vi "FPGA Main.vi"   [LabVIEW 2013]
uses:
  dynamic profibus/profibus master action.ctl
  dynamic profibus/profibus master transmit header.ctl
  dynamic profibus/error enum.ctl
  <vilib>/rvi/eio/common/nirviEmuTemplatePropertySet_errors.vi
  <vilib>/rvi/Emulation/niFpgaSctlEmulationGetInTimedLoop.vi
  <vilib>/rvi/Emulation/niFpgaEmulationReportErrorSimple.vi
  <vilib>/rvi/Emulation/niFpgaGetClockAttributes.vi
  <vilib>/rvi/DataTransferAndStorage/Container/Common/niFpgaContainerExecOnDevCompGetState.vi
  <vilib>/rvi/FIFO/Fifo_Resource/nirvififoEmulationReadFpgaImpl.vi
  <vilib>/rvi/DataTransferAndStorage/Container/Common/niFpgaContainerGetUniqueNameForEmu.vi
  <vilib>/rvi/interface/RandomDataEmulation/nirviRandomDataFPGAFIFO.vi
  <vilib>/rvi/interface/RandomDataEmulation/niFpgaRandomDataHandleErrors.vi
  <vilib>/rvi/eio/common/nirviEmuReportErrorAndStop.vi
  <vilib>/rvi/eio/common/nirviEmuTemplateMethod_errors.vi
  <vilib>/rvi/FIFO/Fifo_Resource/nirvififoEmulationWriteFpgaImpl.vi
  <vilib>/rvi/Emulation/niFpgaCriticalErrorInLSC.vi
  <vilib>/eio/EIOPropertyNode/EIOPropertyNode.xnode
  <vilib>/rvi/DataTransferAndStorage/Container/XNode/niFpgaContainer.xnode
  <vilib>/rvi/FIFO/Fifo_Resource/niFpgaFifoEmulationRefIn.vi
  <vilib>/eio/EIOMethodNode/EIOMethodNode.xnode
  <vilib>/rvi/eio/common/nirviEmuTemplatePropertyGet_errors.vi
  <vilib>/rvi/eio/common/nirviEmuTemplatePropertyGet_noerrors.vi
  <vilib>/rvi/eio/common/nirviEmuTemplatePropertySet_noerrors.vi
  dynamic profibus/dynamic profibus.lvlib
  <vilib>/rvi/LocalResourceManager/LocalResourceManager.xnode
  <vilib>/rvi/DataTransferAndStorage/Register/Emulation/niFpgaRegisterEmulationRefIn.vi
  <vilib>/rvi/DataTransferAndStorage/Container/Common/niFpgaContainerSetEmuInfo.vi
  <vilib>/rvi/DataTransferAndStorage/Register/Emulation/niFpgaRegisterEmulation.vi
types:
  T1 = typedef "dynamic profibus.lvlib/profibus master action.ctl" = enum8{"initialize", "uninitialize", "stop", "get input", "get input size", "set output", "get output size", "get diagnostic", "transfer data", "transfer diagnostics", "read many inputs"}
  T2 = typedef "dynamic profibus.lvlib/profibus master transmit header.ctl" = enum8{"Error", "Input", "Diagnostic", "input size", "output size", "many inputs"}
  T3 = typedef "dynamic profibus.lvlib/error enum.ctl" = u16
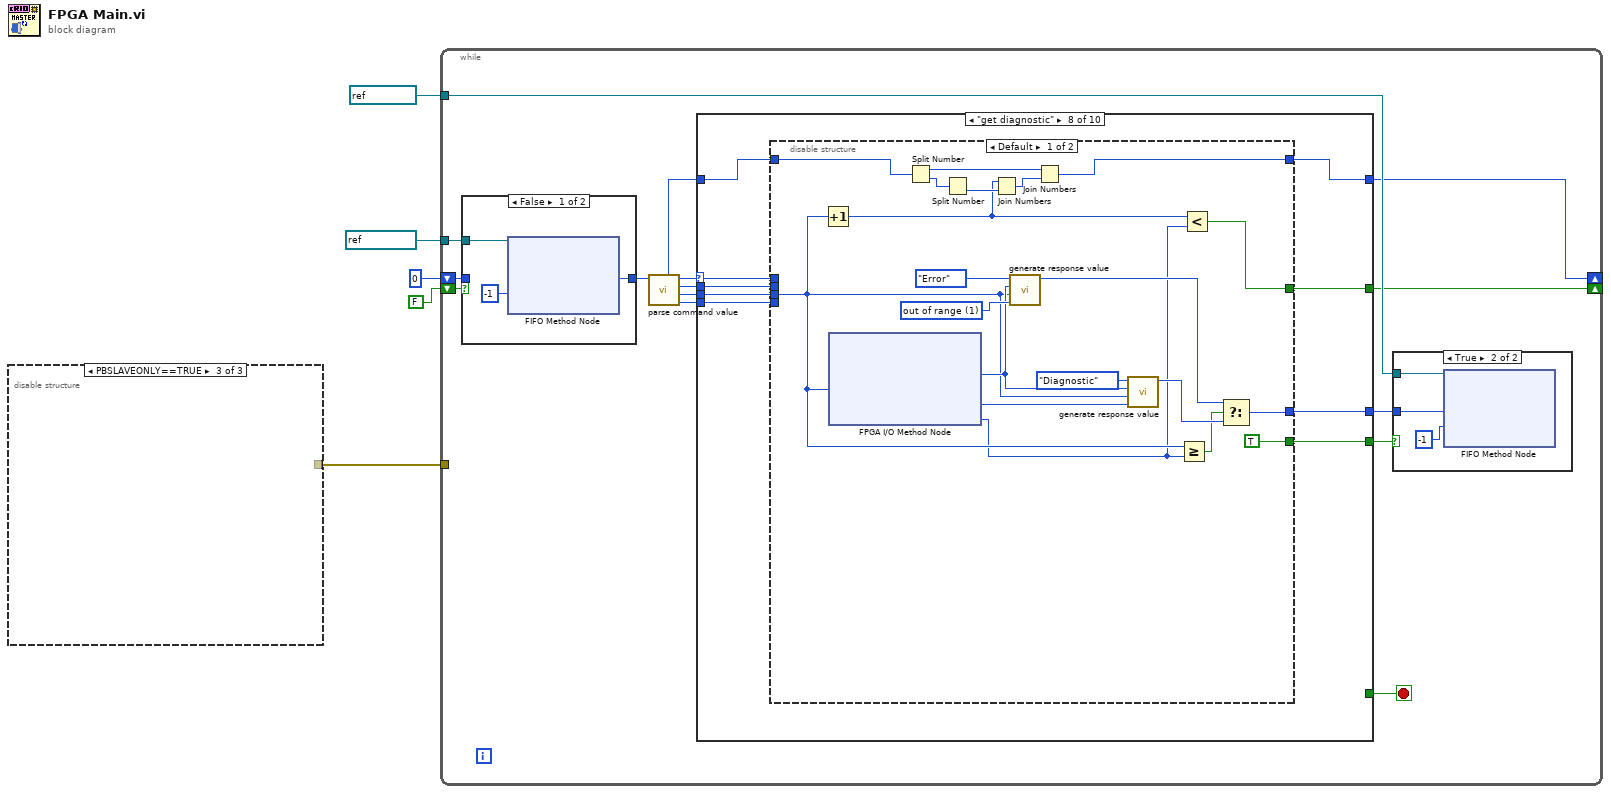
[diagram p0: block diagram]
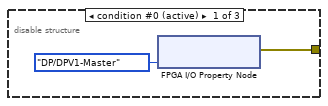
[diagram p2: hidden frame]
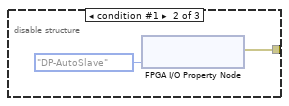
[diagram p3: hidden frame]
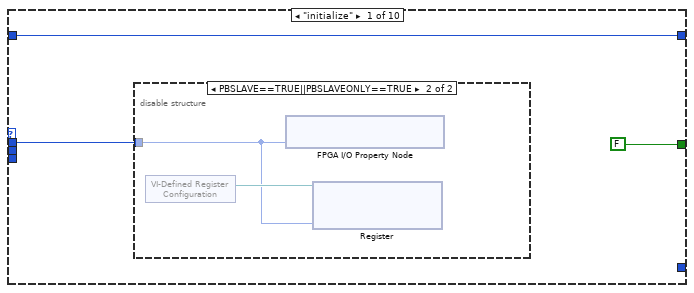
[diagram p6: hidden frame]
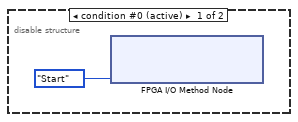
[diagram p7: hidden frame]
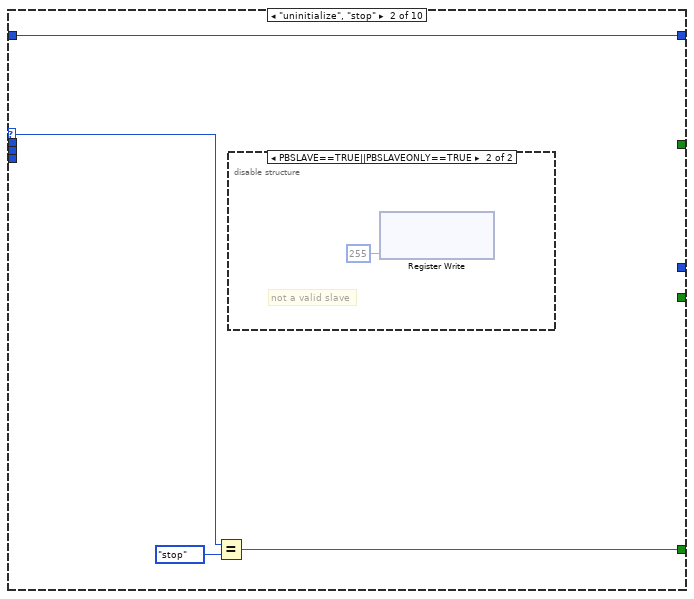
[diagram p8: hidden frame]
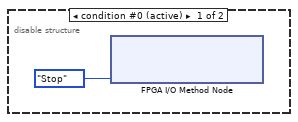
[diagram p9: hidden frame]
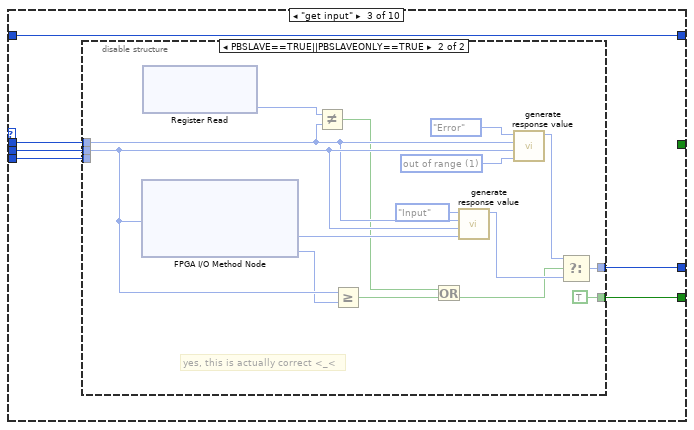
[diagram p10: hidden frame]
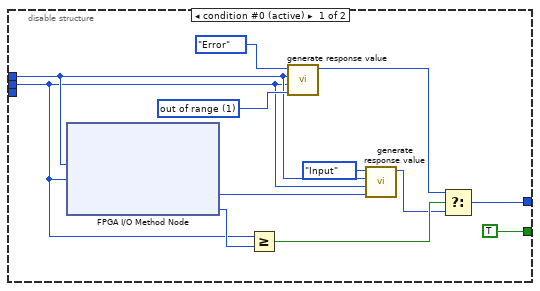
[diagram p11: hidden frame]
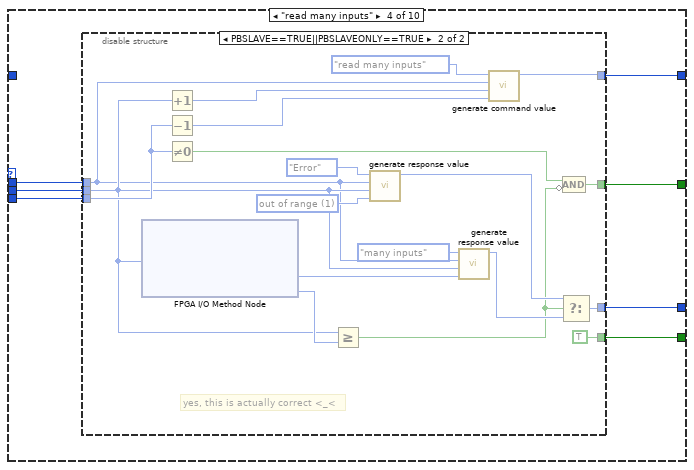
[diagram p12: hidden frame]
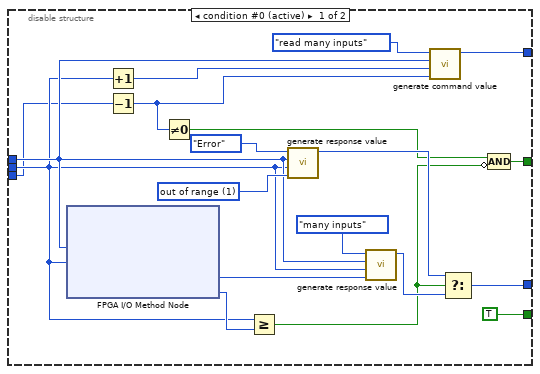
[diagram p13: hidden frame]
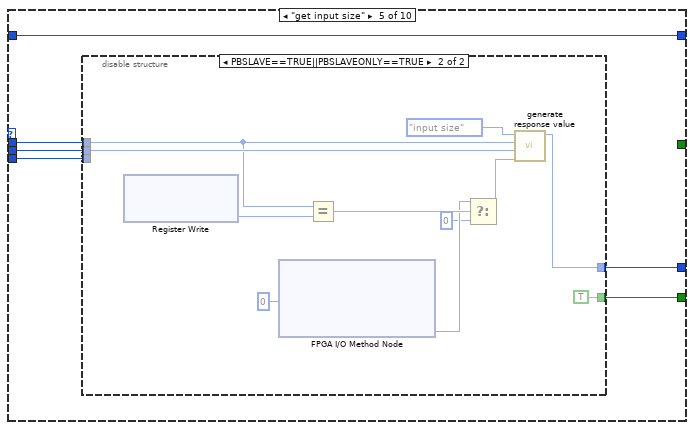
[diagram p14: hidden frame]
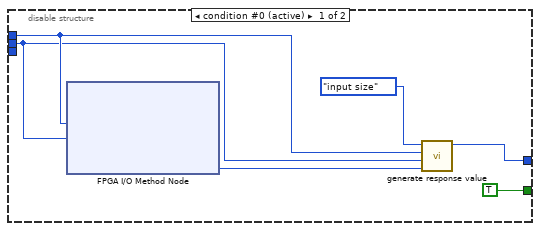
[diagram p15: hidden frame]
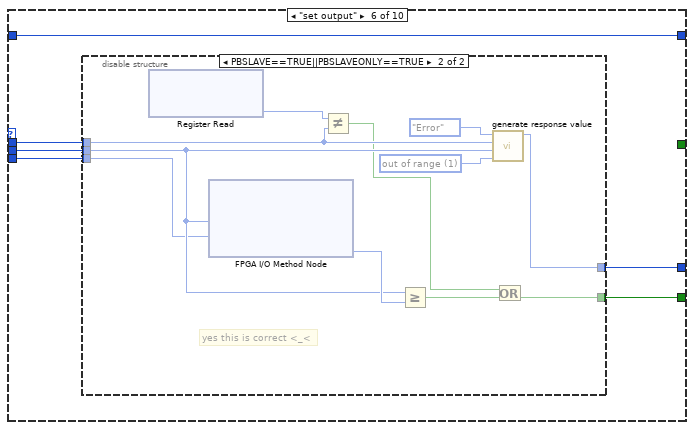
[diagram p16: hidden frame]
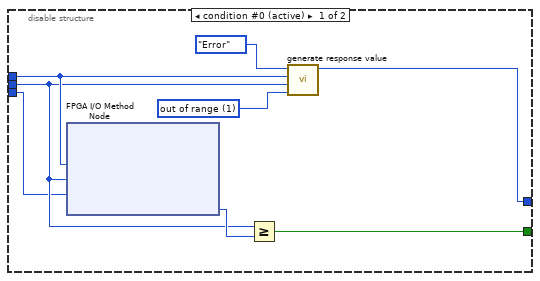
[diagram p17: hidden frame]
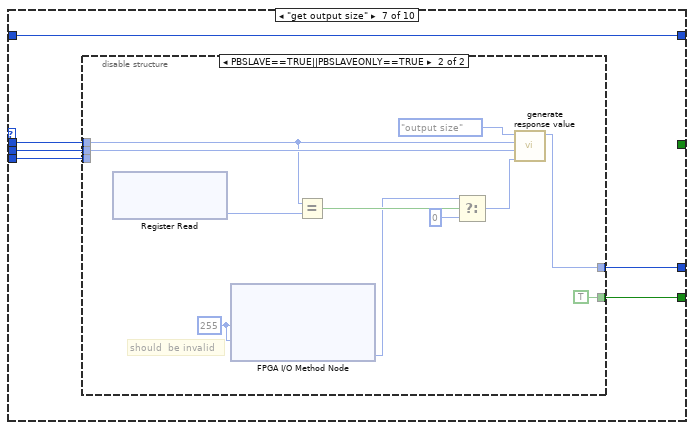
[diagram p18: hidden frame]
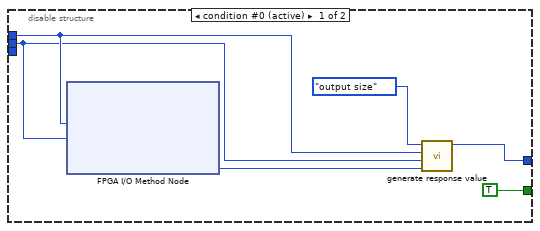
[diagram p19: hidden frame]
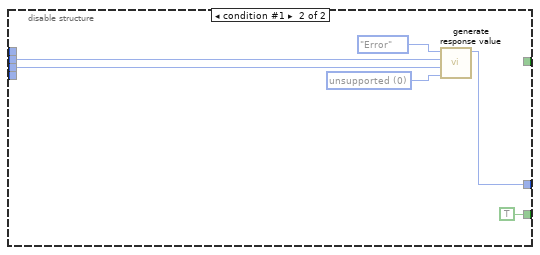
[diagram p20: hidden frame]
diagram:
  n1 = disable-structure shown="PBSLAVEONLY==TRUE" {
    disable-tunnel: [w6 w8 _] -> w3
    frame condition #0 (active) {
      n2 = xnode "FPGA I/O Property Node"("Init cRIO PB"=enum8{"DP/DPV1-Master", "DP-AutoSlave"}."DP/DPV1-Master" ("Start-up cRIO PB")) -> ("error out"=w6:errorcluster)  [unwired: 2 in, 1 out]
    }
    frame condition #1 {
      n3 = xnode "FPGA I/O Property Node"("Init cRIO PB"=enum8{"DP/DPV1-Master", "DP-AutoSlave"}."DP-AutoSlave" ("Start-up cRIO PB")) -> ("error out"=w8:errorcluster)  [unwired: 2 in, 1 out]
    }
    frame condition #2 {
    }
  }
  n4 = while {
    tunnel: refnum<k21> "ToFPGA" ("FIFO In") -> [w23]
    tunnel: refnum<k21> "ToHost" ("FIFO In") -> [w22]
    tunnel: w3 -> [_]
    shift-right: [w10] -> _
    shift-left: FALSE -> [w13]
    shift-right: [w11] -> _
    shift-left: u32 0 ("full element") -> [w12]
    stop <- w24 stop-if-true
    n5 = case shown="False" w13 {
      tunnel: w23 -> [w27 _]
      tunnel: [w26 w28] -> w21
      tunnel: w12 -> [_ w28]
      frame False {
        n6 = xnode ("FIFO Method Node")("Timeout"=-1, "FIFO In"=w27) -> ("Element"=w26:u32)  [unwired: 2 out]
      }
      frame True {
      }
    }
    n7 = call "parse command value.vi"("Element"=w21) -> ("data"=w17:u8, "index"=w18:u8, "device"=w19:u8, "action"=w20:T1, "full element"=w16:u32)  [unwired: 6 in]
    n8 = case shown="\"get diagnostic\"" w20 {
      selector: w20 -> [_ w41 _ _ _ _ _ w195 _ _]
      tunnel: w19 -> [w34 _ w45 w79 w123 w146 w171 w197 w229 w250]
      tunnel: w18 -> [_ _ w49 w83 w127 w150 w175 w201 w233 w254]
      tunnel: w17 -> [_ _ w48 w82 w126 w149 w174 w200 w232 w253]
      tunnel: w16 -> [w33 w38 w44 _ w122 w145 w170 w196 w228 w249]
      tunnel: [_ _ w47 w81 w125 w148 w173 w199 w231 w252] -> w15
      tunnel: [_ _ w46 w80 w124 w147 w172 w198 w230 w251] -> w14
      tunnel: [_ w39 _ _ _ _ _ _ _ _] -> w24
      tunnel: [w33 w38 w44 w78 w122 w145 w170 w194 w228 w249] -> w11
      tunnel: [FALSE _ _ w77 _ _ _ w193 _ _] -> w10
      frame "initialize" {
        n9 = disable-structure shown="PBSLAVE==TRUE||PBSLAVEONLY==TRUE" {
          disable-tunnel: w34 -> [_ w36]
          frame condition #0 (active) {
            n10 = xnode "FPGA I/O Method Node"("Mode"=enum16{"Start", "Stop"}."Start") -> ()  [unwired: 2 in, 2 out]
          }
          frame condition #1 {
            n11 = xnode ("VI-Defined Register Configuration")() -> ("Register Out"=w37:refnum<k21>)
            n12 = xnode "FPGA I/O Property Node"("DP-AutoSlave Address"=w36) -> ()  [unwired: 2 in, 2 out]
            n13 = xnode "Register"("Data"=w36, "Register In"=w37) -> ()  [unwired: 1 out]
          }
        }
      }
      frame "uninitialize", "stop" {
        n14 = Equal?(x=w41, y=profibus_master_action."stop") -> (x = y?=w39:bool)
        n15 = disable-structure shown="PBSLAVE==TRUE||PBSLAVEONLY==TRUE" {
          frame condition #0 (active) {
            n16 = xnode "FPGA I/O Method Node"("Mode"=enum16{"Start", "Stop"}."Stop") -> ()  [unwired: 2 in, 2 out]
          }
          frame condition #1 {
            # "not a valid slave"
            n17 = xnode "Register Write"("Data"=u8 255) -> ()  [unwired: 1 in, 1 out]
          }
        }
      }
      frame "get input" {
        n18 = disable-structure shown="PBSLAVE==TRUE||PBSLAVEONLY==TRUE" {
          disable-tunnel: w49 -> [w51 w67]
          disable-tunnel: w48 -> [_ _]
          disable-tunnel: [TRUE TRUE] -> w47
          disable-tunnel: [w55 w68] -> w46
          disable-tunnel: w45 -> [w52 w64]
          frame condition #0 (active) {
            w59 = T3 1 items=["unsupported", "out of range"]
            n19 = xnode "FPGA I/O Method Node"("Slave"=w52, "Index"=w51) -> ("Data"=w53:u8, "Length"=w58:u8)  [unwired: 1 in, 1 out]
            n20 = Greater Or Equal?(x=w51, y=w58) -> (x >= y?=w57:bool)
            n21 = call "generate response value.vi"("data"=w59, "index"=w51, "device"=w52, "header"=profibus_master_transmit_header."Error") -> ("Element"=w56:u32)  [unwired: 7 in]
            n22 = call "generate response value.vi"("data"=w53, "index"=w51, "device"=w52, "header"=profibus_master_transmit_header."Input") -> ("Element"=w54:u32)  [unwired: 7 in]
            n23 = Select(t=w56, s=w57, f=w54) -> (s? t:f=w55:u32)
          }
          frame condition #1 {
            w71 = T3 1 items=["unsupported", "out of range"]
            # "yes, this is actually correct <_<"
            n24 = xnode "FPGA I/O Method Node"("Index"=w67) -> ("Data"=w72:u8, "Length"=w66:u8)  [unwired: 1 in, 1 out]
            n25 = xnode "Register Read"() -> ("Data"=w63:u8)  [unwired: 1 in, 1 out]
            n26 = Not Equal?(x=w63, y=w64) -> (x != y?=w62:bool)
            n27 = Greater Or Equal?(x=w67, y=w66) -> (x >= y?=w75:bool)
            n28 = Or(x=w62, y=w75) -> (x .or. y?=w65:bool)
            n29 = call "generate response value.vi"("data"=w72, "index"=w67, "device"=w64, "header"=profibus_master_transmit_header."Input") -> ("Element"=w76:u32)  [unwired: 7 in]
            n30 = call "generate response value.vi"("data"=w71, "index"=w67, "device"=w64, "header"=profibus_master_transmit_header."Error") -> ("Element"=w74:u32)  [unwired: 7 in]
            n31 = Select(t=w74, s=w65, f=w76) -> (s? t:f=w68:u32)
          }
        }
      }
      frame "read many inputs" {
        n32 = disable-structure shown="PBSLAVE==TRUE||PBSLAVEONLY==TRUE" {
          disable-tunnel: w83 -> [w90 w106]
          disable-tunnel: w82 -> [w87 w107]
          disable-tunnel: [TRUE TRUE] -> w81
          disable-tunnel: [w97 w114] -> w80
          disable-tunnel: w79 -> [w91 w105]
          disable-tunnel: [w93 w108] -> w78
          disable-tunnel: [w85 w104] -> w77
          frame condition #0 (active) {
            w100 = T3 1 items=["unsupported", "out of range"]
            n33 = xnode "FPGA I/O Method Node"("Slave"=w91, "Index"=w90) -> ("Data"=w95:u8, "Length"=w99:u8)  [unwired: 1 in, 1 out]
            n34 = Increment(x=w90) -> (x+1=w89:u8)
            n35 = Decrement(x=w87) -> (x-1=w84:u8)
            n36 = Not Equal To 0?(x=w84) -> (x != 0?=w86:bool)
            n37 = Greater Or Equal?(x=w90, y=w99) -> (x >= y?=w88:bool)
            n38 = call "generate response value.vi"("data"=w100, "index"=w90, "device"=w91, "header"=profibus_master_transmit_header."Error") -> ("Element"=w98:u32)  [unwired: 7 in]
            n39 = call "generate response value.vi"("data"=w95, "index"=w90, "device"=w91, "header"=profibus_master_transmit_header."many inputs") -> ("Element"=w96:u32)  [unwired: 7 in]
            n40 = call "generate command value.vi"("data"=w84, "index"=w89, "device"=w91, "action"=profibus_master_action."read many inputs") -> ("Element"=w93:u32)  [unwired: 7 in]
            n41 = Select(t=w98, s=w88, f=w96) -> (s? t:f=w97:u32)
            n42 = Compound Arithmetic op=AND(w86, invert w88) -> (w85:bool)
          }
          frame condition #1 {
            w117 = T3 1 items=["unsupported", "out of range"]
            # "yes, this is actually correct <_<"
            n43 = xnode "FPGA I/O Method Node"("Index"=w106) -> ("Data"=w118:u8, "Length"=w113:u8)  [unwired: 1 in, 1 out]
            n44 = Increment(x=w106) -> (x+1=w111:u8)
            n45 = Decrement(x=w107) -> (x-1=w110:u8)
            n46 = Not Equal To 0?(x=w107) -> (x != 0?=w109:bool)
            n47 = Greater Or Equal?(x=w106, y=w113) -> (x >= y?=w103:bool)
            n48 = call "generate response value.vi"("data"=w117, "index"=w106, "device"=w105, "header"=profibus_master_transmit_header."Error") -> ("Element"=w120:u32)  [unwired: 7 in]
            n49 = call "generate response value.vi"("data"=w118, "index"=w106, "device"=w105, "header"=profibus_master_transmit_header."many inputs") -> ("Element"=w121:u32)  [unwired: 7 in]
            n50 = call "generate command value.vi"("data"=w110, "index"=w111, "device"=w105, "action"=profibus_master_action."read many inputs") -> ("Element"=w108:u32)  [unwired: 7 in]
            n51 = Select(t=w120, s=w103, f=w121) -> (s? t:f=w114:u32)
            n52 = Compound Arithmetic op=AND(w109, invert w103) -> (w104:bool)
          }
        }
      }
      frame "get input size" {
        n53 = disable-structure shown="PBSLAVE==TRUE||PBSLAVEONLY==TRUE" {
          disable-tunnel: w127 -> [w128 w139]
          disable-tunnel: w126 -> [_ _]
          disable-tunnel: [TRUE TRUE] -> w125
          disable-tunnel: [w131 w143] -> w124
          disable-tunnel: w123 -> [w129 w138]
          frame condition #0 (active) {
            n54 = xnode "FPGA I/O Method Node"("Slave"=w129, "Index"=w128) -> ("Length"=w130:u8)  [unwired: 1 in, 2 out]
            n55 = call "generate response value.vi"("data"=w130, "index"=w128, "device"=w129, "header"=profibus_master_transmit_header."input size") -> ("Element"=w131:u32)  [unwired: 7 in]
          }
          frame condition #1 {
            n56 = xnode "Register Write"() -> ("Data"=w140:u8)  [unwired: 1 in, 1 out]
            n57 = xnode "FPGA I/O Method Node"("Index"=u8 0) -> ("Length"=w136:u8)  [unwired: 1 in, 2 out]
            n58 = Equal?(x=w138, y=w140) -> (x = y?=w137:bool)
            n59 = Select(t=w136, s=w137, f=u8 0) -> (s? t:f=w134:u8)
            n60 = call "generate response value.vi"("data"=w134, "index"=w139, "device"=w138, "header"=profibus_master_transmit_header."input size") -> ("Element"=w143:u32)  [unwired: 7 in]
          }
        }
      }
      frame "set output" {
        n61 = disable-structure shown="PBSLAVE==TRUE||PBSLAVEONLY==TRUE" {
          disable-tunnel: w150 -> [w154 w164]
          disable-tunnel: w149 -> [w153 w163]
          disable-tunnel: [w152 w162] -> w148
          disable-tunnel: [w151 w165] -> w147
          disable-tunnel: w146 -> [w155 w160]
          frame condition #0 (active) {
            w157 = T3 1 items=["unsupported", "out of range"]
            n62 = xnode "FPGA I/O Method Node"("Slave"=w155, "Index"=w154, "Data"=w153) -> ("Length"=w156:u8)  [unwired: 1 in, 1 out]
            n63 = Greater Or Equal?(x=w154, y=w156) -> (x >= y?=w152:bool)
            n64 = call "generate response value.vi"("data"=w157, "index"=w154, "device"=w155, "header"=profibus_master_transmit_header."Error") -> ("Element"=w151:u32)  [unwired: 7 in]
          }
          frame condition #1 {
            w168 = T3 1 items=["unsupported", "out of range"]
            # "yes this is correct <_<"
            n65 = xnode "Register Read"() -> ("Data"=w161:u8)  [unwired: 1 in, 1 out]
            n66 = xnode "FPGA I/O Method Node"("Index"=w164, "Data"=w163) -> ("Length"=w169:u8)  [unwired: 1 in, 1 out]
            n67 = Not Equal?(x=w161, y=w160) -> (x != y?=w159:bool)
            n68 = Greater Or Equal?(x=w164, y=w169) -> (x >= y?=w166:bool)
            n69 = call "generate response value.vi"("data"=w168, "index"=w164, "device"=w160, "header"=profibus_master_transmit_header."Error") -> ("Element"=w165:u32)  [unwired: 7 in]
            n70 = Or(x=w159, y=w166) -> (x .or. y?=w162:bool)
          }
        }
      }
      frame "get output size" {
        n71 = disable-structure shown="PBSLAVE==TRUE||PBSLAVEONLY==TRUE" {
          disable-tunnel: w175 -> [w176 w189]
          disable-tunnel: w174 -> [_ _]
          disable-tunnel: [TRUE TRUE] -> w173
          disable-tunnel: [w179 w191] -> w172
          disable-tunnel: w171 -> [w177 w182]
          frame condition #0 (active) {
            n72 = xnode "FPGA I/O Method Node"("Slave"=w177, "Index"=w176) -> ("Length"=w178:u8)  [unwired: 1 in, 2 out]
            n73 = call "generate response value.vi"("data"=w178, "index"=w176, "device"=w177, "header"=profibus_master_transmit_header."output size") -> ("Element"=w179:u32)  [unwired: 7 in]
          }
          frame condition #1 {
            w188 = u8 255 ("Index")
            # "should  be invalid"
            n74 = xnode "Register Read"() -> ("Data"=w187:u8)  [unwired: 1 in, 1 out]
            n75 = xnode "FPGA I/O Method Node"("Index"=w188, "Data"=w188) -> ("Length"=w184:u8)  [unwired: 1 in, 1 out]
            n76 = Equal?(x=w182, y=w187) -> (x = y?=w186:bool)
            n77 = Select(t=w184, s=w186, f=u8 0) -> (s? t:f=w183:u8)
            n78 = call "generate response value.vi"("data"=w183, "index"=w189, "device"=w182, "header"=profibus_master_transmit_header."output size") -> ("Element"=w191:u32)  [unwired: 7 in]
          }
        }
      }
      frame "get diagnostic" {
        n79 = disable-structure shown="Default" {
          disable-tunnel: w201 -> [w211 w224]
          disable-tunnel: w200 -> [_ _]
          disable-tunnel: [TRUE TRUE] -> w199
          disable-tunnel: [w217 w225] -> w198
          disable-tunnel: w197 -> [_ w223]
          disable-tunnel: w196 -> [w210 _]
          disable-tunnel: w195 -> [_ _]
          disable-tunnel: [w205 _] -> w194
          disable-tunnel: [w202 _] -> w193
          frame condition #0 (active) {
            w219 = T3 1 items=["unsupported", "out of range"]
            n80 = Increment(x=w211) -> (x+1=w203:u8)
            n81 = xnode "FPGA I/O Method Node"("Index"=w211) -> ("Slave"=w213:i8, "Data"=w215:u8, "Length"=w204:u8)  [unwired: 1 in, 1 out]
            n82 = Split Number(x=w210) -> (hi(x)=w206:u16, lo(x)=w209:u16)
            n83 = Split Number(x=w209) -> (lo(x)=w208:u8)  [unwired: 1 out]
            n84 = Join Numbers(hi=w203, lo=w208) -> ((hi.lo)=w207:u16)
            n85 = call "generate response value.vi"("data"=w219, "index"=w211, "device"=w213, "header"=profibus_master_transmit_header."Error") -> ("Element"=w218:u32)  [unwired: 7 in]
            n86 = Join Numbers(hi=w206, lo=w207) -> ((hi.lo)=w205:u32)
            n87 = call "generate response value.vi"("data"=w215, "index"=w211, "device"=w213, "header"=profibus_master_transmit_header."Diagnostic") -> ("Element"=w216:u32)  [unwired: 7 in]
            n88 = Greater Or Equal?(x=w211, y=w204) -> (x >= y?=w212:bool)
            n89 = Less?(x=w203, y=w204) -> (x < y?=w202:bool)
            n90 = Select(t=w218, s=w212, f=w216) -> (s? t:f=w217:u32)
          }
          frame condition #1 {
            w226 = T3 0 items=["unsupported", "out of range"]
            n91 = call "generate response value.vi"("data"=w226, "index"=w224, "device"=w223, "header"=profibus_master_transmit_header."Error") -> ("Element"=w225:u32)  [unwired: 7 in]
          }
        }
      }
      frame "transfer data" {
        n92 = disable-structure shown="Default" {
          disable-tunnel: w233 -> [w237 w246]
          disable-tunnel: w232 -> [_ _]
          disable-tunnel: [w236 w240] -> w231
          disable-tunnel: [w235 w247] -> w230
          disable-tunnel: w229 -> [w238 w245]
          frame condition #0 (active) {
            n93 = xnode "FPGA I/O Method Node"("Slave"=w238) -> ("Slave Status"=w234:u8)  [unwired: 1 in, 1 out]
            n94 = Not Equal To 0?(x=w234) -> (x != 0?=w236:bool)
            n95 = call "generate response value.vi"("data"=w234, "index"=w237, "device"=w238, "header"=profibus_master_transmit_header."Error") -> ("Element"=w235:u32)  [unwired: 7 in]
          }
          frame condition #1 {
            # "bit 7 = valid"
            n96 = xnode "FPGA I/O Method Node"() -> ("Slave Status"=w244:u8)  [unwired: 1 in, 2 out]
            n97 = Number To Boolean Array(number=w244) -> (Boolean array=w243:bool[])
            n98 = Index Array(array=w243, index=7) -> (element=w241:bool)
            n99 = call "generate response value.vi"("data"=w244, "index"=w246, "device"=w245, "header"=profibus_master_transmit_header."Error") -> ("Element"=w247:u32)  [unwired: 7 in]
            n100 = Not(x=w241) -> (.not. x?=w240:bool)
          }
        }
      }
      frame "transfer diagnostics" {
        n101 = disable-structure shown="Default" {
          disable-tunnel: w254 -> [w256 w262]
          disable-tunnel: w253 -> [_ _]
          disable-tunnel: [w258 _] -> w252
          disable-tunnel: [w257 w263] -> w251
          disable-tunnel: w250 -> [w255 w261]
          frame condition #0 (active) {
            n102 = xnode "FPGA I/O Method Node"("Slave"=w255) -> ("Slave Status"=w259:u8)  [unwired: 1 in, 2 out]
            n103 = Not Equal To 0?(x=w259) -> (x != 0?=w258:bool)
            n104 = call "generate response value.vi"("data"=w259, "index"=w256, "device"=w255, "header"=profibus_master_transmit_header."Error") -> ("Element"=w257:u32)  [unwired: 7 in]
          }
          frame condition #1 {
            w264 = T3 0 items=["unsupported", "out of range"]
            n105 = call "generate response value.vi"("data"=w264, "index"=w262, "device"=w261, "header"=profibus_master_transmit_header."Error") -> ("Element"=w263:u32)  [unwired: 7 in]
          }
        }
      }
    }
    n106 = case shown="True" w15 {
      tunnel: w22 -> [_ w30]
      tunnel: w14 -> [_ w29]
      frame False {
      }
      frame True {
        n107 = xnode ("FIFO Method Node")("Element"=w29, "Timeout"=-1, "FIFO In"=w30) -> ()  [unwired: 2 out]
      }
    }
  }
